vi "0003_FireAt1015SpecificYear.vi"(8 "error in (no error)":errorcluster) -> (0 "error out":errorcluster)   [LabVIEW 2013]
uses:
  <vilib>/addons/_JKI Toolkits/Caraya/classes/Assert/Assert True.vi
  source/Cron/Create Cron Expression.vi
  source/Cron/Compute Next Cron.vi
  source/Cron.Quartz/Cron.Quartz.lvclass
  <vilib>/addons/_JKI Toolkits/Caraya/classes/Test/Test.lvclass
  <vilib>/addons/_JKI Toolkits/Caraya/classes/Assert/Assert.lvclass
  source/openCron.lvlib
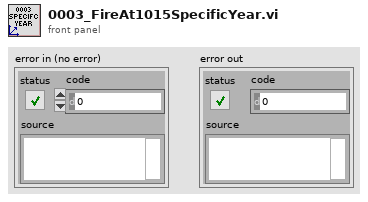
[diagram p1: front panel]
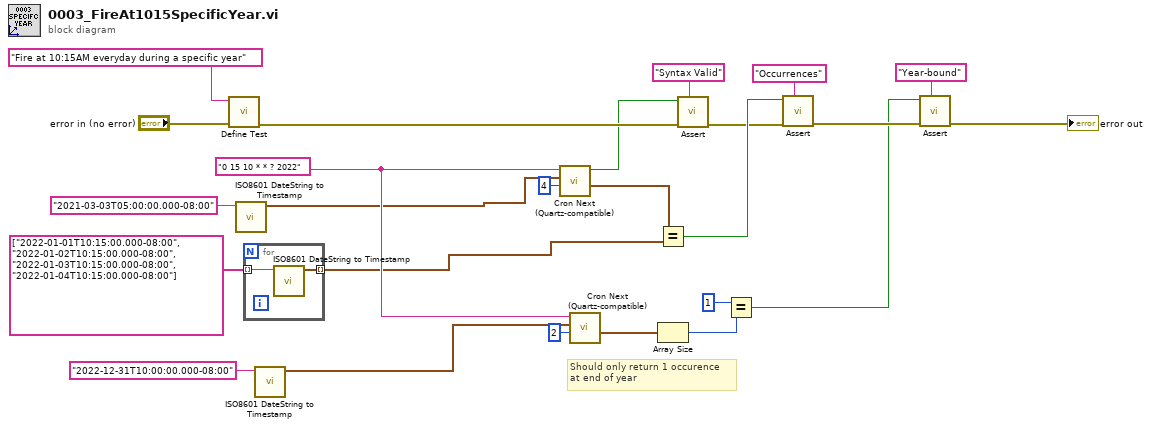
[diagram p0: block diagram]
diagram:
  w12 = "0 15 10 * * ? 2022" ("Expression")
  # "Should only return 1 occurence\nat end of year"
  n1 = call <vilib>:"Define Test.vi"("error in (no error)"="error in (no error)", "Label (VI Title)"="Fire at 10:15AM everyday during a specific year") -> ("error out"=w23:errorcluster)  [unwired: 8 in, 1 out]
  n2 = call <vilib>:"ISO8601 DateString to Timestamp.vi"("ISO8601 Date String"="2021-03-03T05:00:00.000-08:00" ("Expression")) -> ("Timestamp"=w3:timestamp)  [unwired: 8 in, 2 out]
  n3 = for {
    tunnel: string[] ["2022-01-01T10:15:00.000-08:00", "2022-01-02T10:15:00.000-08:00", "2022-01-03T10:15:00.000-08:00", "2022-01-04T10:15:00.000-08:00"] -> [w27] mode=indexing
    tunnel: [w26] -> w2 mode=indexing
    n4 = call <vilib>:"ISO8601 DateString to Timestamp.vi"("ISO8601 Date String"=w27) -> ("Timestamp"=w26:timestamp)  [unwired: 8 in, 2 out]
  }
  n5 = call <vilib>:"ISO8601 DateString to Timestamp.vi"("ISO8601 Date String"="2022-12-31T10:00:00.000-08:00" ("Expression")) -> ("Timestamp"=w1:timestamp)  [unwired: 8 in, 2 out]
  n6 = call "Cron Next (Quartz-compatible).vi"("Nb Occurences (min: 1)"=u16 4, "Reference timestamp (Now)"=w3, "Cron Expression"=w12) -> ("Occurences"=w19:timestamp[], "syntax valid?"=w20:bool)  [unwired: 6 in, 1 out]
  n7 = call "Cron Next (Quartz-compatible).vi"("Nb Occurences (min: 1)"=u16 2, "Reference timestamp (Now)"=w1, "Cron Expression"=w12) -> ("Occurences"=w10:timestamp[])  [unwired: 6 in, 2 out]
  n8 = Equal?(x=w19, y=w2) -> (x = y?=w22:bool)
  n9 = Array Size(array=w10) -> (size(s)=w9:i32)
  n10 = call-poly <vilib>:"Assert.vi"("Label"="Syntax Valid" ("Label (VI Title)"), "error in (no error)"=w23, "True?"=w20) -> ("error out"=w21:errorcluster)  [unwired: 7 in, 1 out]
  n11 = Equal?(x=1, y=w9) -> (x = y?=w7:bool)
  n12 = call-poly <vilib>:"Assert.vi"("Label"="Occurrences" ("Label (VI Title)"), "error in (no error)"=w21, "True?"=w22) -> ("error out"=w14:errorcluster)  [unwired: 7 in, 1 out]
  n13 = call-poly <vilib>:"Assert.vi"("Label"="Year-bound" ("Label (VI Title)"), "error in (no error)"=w14, "True?"=w7) -> ("error out"=→"error out":errorcluster)  [unwired: 7 in, 1 out]
